vi "Apply Config.vi"(8 "Error In":errorcluster, 10 "Name":string, 11 "TopModule In":refnum<class "TopModule.lvclass">) -> (0 "Error Out":errorcluster, 3 "TopModule Out":refnum<class "TopModule.lvclass">)   [LabVIEW 2020, in "TopModule.lvclass"]
uses:
  TopModule.lvclass
  TopModule.lvclass/TopModule.ctl
  IConfig/IConfig.lvclass
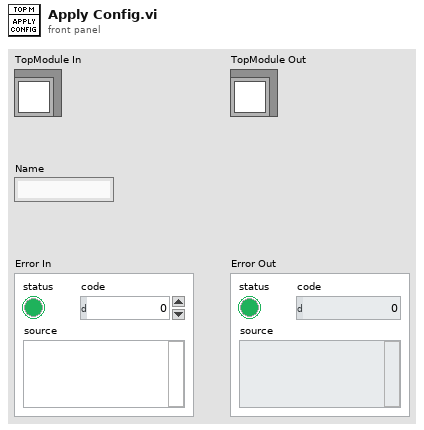
[diagram p1: front panel]
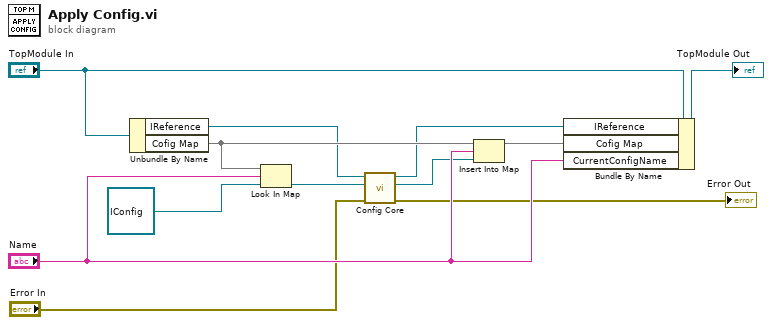
[diagram p0: block diagram]
diagram:
  n1 = Unbundle By Name("TopModule In") -> ("IReference"=w6:refnum<class "IRef.lvclass">, "Cofig Map"=w9:map{string, refnum<class "IConfig.lvclass">})
  n2 = Look In Map(map=w9, key="Name", default value=refnum<class "IConfig.lvclass"> refnum ("IConfig.lvclass")) -> (value=w5:refnum<class "IConfig.lvclass">)  [unwired: 1 out]
  n3 = call-dynamic "Config Core.vi"("Error In"="Error In", "IConfig In"=w5, "Hardware In"=w6) -> ("Error Out"=→"Error Out":errorcluster, "IConfig Out"=w2:refnum<class "IConfig.lvclass">, "Hardware Out"=w3:refnum<class "IRef.lvclass">)  [unwired: 6 in]
  n4 = Insert Into Map(map in=w9, key="Name", value=w2) -> (map out=w8:map{string, refnum<class "IConfig.lvclass">})  [unwired: 2 out]
  n5 = Bundle By Name(cluster="TopModule In", "IReference"=w3, "Cofig Map"=w8, "CurrentConfigName"="Name") -> (→"TopModule Out":refnum<class "TopModule.lvclass">)
